vi "Deserialize Picture Control Data.vi"(8 "error in":errorcluster, 11 "Layers in":refnum<class "Layer.lvclass">[](array[class])) -> (0 "error out":errorcluster, 3 "Layers out":refnum<class "Layer.lvclass">[](array[class]))   [LabVIEW 2020, in "lv_icon.lvlib"]
doc: "Every concentenate picture adds more and more data to the picture, therefore\nhis process is used to keep the picture memory amount as low as possible."
uses:
  lv_icon.lvlib
  Classes/Layer/Layer.lvclass
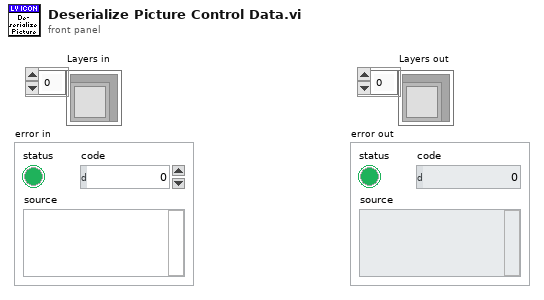
[diagram p1: front panel]
types:
  T1 = typedef "Layer.ctl" = cluster{"LayerIcon":picture, "LayerName":string, "Opacity":u8, "Visibility?":bool}
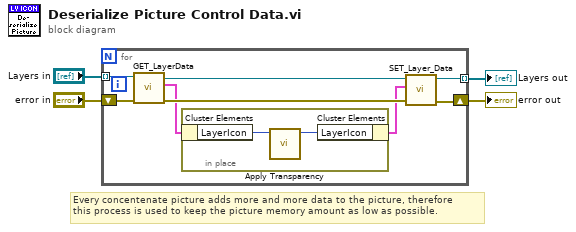
[diagram p0: block diagram]
diagram:
  # "Every concentenate picture adds more and more data to the picture, therefore\nthis process is used to keep the picture memory amount as low as possible."
  n1 = for {
    tunnel: "Layers in" -> [w9] mode=indexing
    tunnel: [w7] -> w1 mode=indexing
    shift-right: [w10] -> w3
    shift-left: "error in" -> [w12]
    n2 = call-dynamic "GET_LayerData.vi"("error in (no error)"=w12, "Layer.lvclass in"=w9) -> ("error out"=w11:errorcluster, "Data"=w6:T1, "Layer.lvclass out"=w8:refnum<class "Layer.lvclass">)  [unwired: 7 out]
    n3 = in-place {
      n4 = in-place-cluster #1(w6) -> ("LayerIcon"=w14:picture)
      n5 = call "Apply Transparency.vi"("in"=w14) -> ("out"=w13:picture)  [unwired: 1 in, 9 out]
      n6 = in-place-cluster #1("LayerIcon"=w13) -> (w5:T1)
    }
    n7 = call-dynamic "SET_Layer_Data.vi"("error in (no error)"=w11, "Data"=w5, "Layer.lvclass in"=w8) -> ("error out"=w10:errorcluster, "Layer.lvclass out"=w7:refnum<class "Layer.lvclass">)  [unwired: 1 in, 6 out]
  }
  "Layers out" <- w1
  "error out" <- w3
